vi "variant to bool.vi"(1 "Variant":variant) -> (0 "Boolean":bool)   [LabVIEW 2025]
doc: "convert variant data to a LabVIEW Boolean\n<B>Input:</B>\nVariant (skalar)\n<B>Output:</B>\nBoolean"
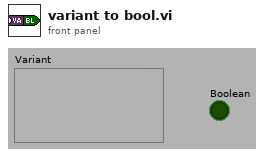
[diagram p1: front panel]
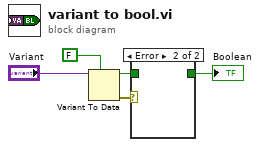
[diagram p0: block diagram]
diagram:
  n1 = Variant To Data(type=FALSE, Variant="Variant") -> (data=w4:bool, error out=w5:errorcluster)  [unwired: 1 in]
  n2 = case shown="Error" w5 {
    tunnel: w4 -> [w6 _]
    tunnel: [w6 _] -> w2
    frame No Error {
    }
    frame Error {
    }
  }
  "Boolean" <- w2
